vi "change channel select data typel test.vi"() -> ()   [LabVIEW 2015, in "tag select module tests.lvlib"]
uses:
  tag select module tests.lvlib
  module/configuration/tag select configuration.ctl
  <vilib>/NI/Tag Bus Module Framework/channel/TBM channel.lvclass
  <vilib>/NI/Tag Bus/tag/Data Type.ctl
  module/configuration/tag select module configuration.lvclass/tag select module configuration.ctl
  <vilib>/NI/Tag Bus/tag/tag descriptor.lvclass/tag descriptor.ctl
  module/configuration/Read tag select.vi
  <vilib>/NI/Tag Bus/tag/tag descriptor.lvclass
  module/configuration/tag select module configuration.lvclass
panel:
  out "data type 2":T1
  out "data type":T1
  out "data output 2":T1
  out "data select 2":T1
  out "data input A 2":T1
  out "data Input B 2":T1
  out "data Input B":T1
  out "data input A":T1
  out "data select":T1
  out "data output":T1
  out "input A 2":string
  out "input B 2":string
  out "input A":string
  out "input B":string
  out "select 2":string
  out "output 2":string
  out "select":string
  out "output":string
  out "tag select 2":T2[](array[typedef])
  out "tag select":T2[](array[typedef])
  out "no err":errorcluster
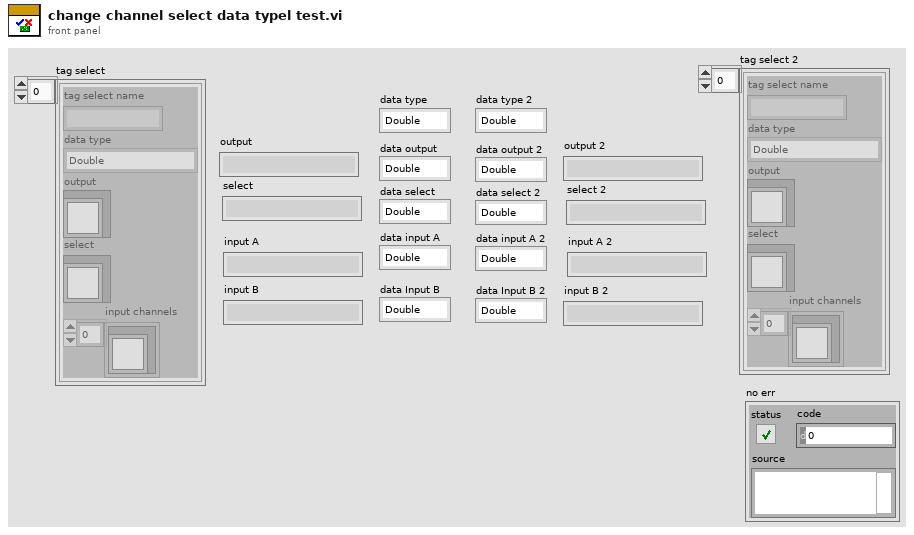
[diagram p1: front panel]
types:
  T1 = typedef "tag bus.lvlib/tag descriptor.lvclass/Data Type.ctl" = enum16{"Double", "Single", "I64", "I32", "I16", "I8", "U64", "U32", "U16", "U8", "Boolean", "String", "Array of Double", "Array of Single", "Array of I64", "Array of I32", "Array of I16", "Array of I8", "Array of U64", "Array of U32", "Array of U16", "Array of U8", "Array of Boolean", "Array of String"}
  T2 = typedef "tag select module configuration.lvclass/tag select configuration.ctl" = cluster{"tag select name":string, "data type":T1, "output":refnum<class "TBM channel.lvclass">, "select":refnum<class "TBM channel.lvclass">, "input channels":refnum<class "TBM channel.lvclass">[]}
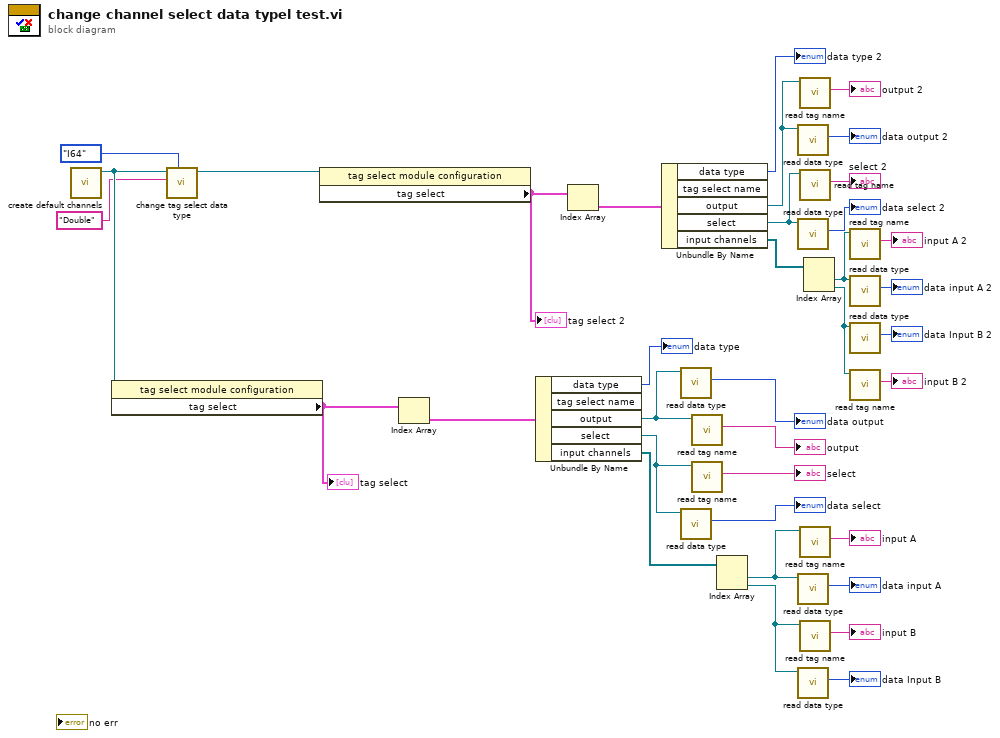
[diagram p0: block diagram]
diagram:
  n1 = call "create default channels.vi"() -> ("module"=w6:refnum<class "tag select module configuration.lvclass">)  [unwired: 8 in, 3 out]
  n2 = property class="tag select module configuration"(reference=w6) -> ("tag select"=w36:T2[])  [unwired: 1 in, 2 out]
  "tag select" <- w36
  n3 = call "change tag select data type.vi"("data type"=Data_Type."I64", "tag select name"="Double" ("old name"), "tag select  module configuration in"=w6) -> ("tag select module configuration out"=w5:refnum<class "tag select module configuration.lvclass">)  [unwired: 6 in, 2 out]
  n4 = property class="tag select module configuration"(reference=w5) -> ("tag select"=w29:T2[])  [unwired: 1 in, 2 out]
  "tag select 2" <- w29
  n5 = Index Array(array=w36) -> (element=w35:T2)  [unwired: 1 in]
  n6 = Unbundle By Name(w35) -> ("data type"=→"data type":T1, "output"=w15:refnum<class "TBM channel.lvclass">, "select"=w16:refnum<class "TBM channel.lvclass">, "input channels"=w28:refnum<class "TBM channel.lvclass">[])  [unwired: 1 out]
  n7 = Index Array(array=w29) -> (element=w32:T2)  [unwired: 1 in]
  n8 = Unbundle By Name(w32) -> ("data type"=→"data type 2":T1, "output"=w10:refnum<class "TBM channel.lvclass">, "select"=w9:refnum<class "TBM channel.lvclass">, "input channels"=w23:refnum<class "TBM channel.lvclass">[])  [unwired: 1 out]
  n9 = call <vilib>:"read data type.vi"("system tag in"=w15) -> ("data type"=→"data output":T1)  [unwired: 8 in, 2 out]
  n10 = call <vilib>:"read data type.vi"("system tag in"=w16) -> ("data type"=→"data select":T1)  [unwired: 8 in, 2 out]
  n11 = call <vilib>:"read tag name.vi"("system tag in"=w15) -> ("name"=→"output":string)  [unwired: 8 in, 2 out]
  n12 = call <vilib>:"read tag name.vi"("system tag in"=w16) -> ("name"=→"select":string)  [unwired: 8 in, 2 out]
  n13 = Index Array(array=w28) -> (element #1=w17:refnum<class "TBM channel.lvclass">, element #2=w18:refnum<class "TBM channel.lvclass">)  [unwired: 2 in]
  n14 = call <vilib>:"read data type.vi"("system tag in"=w10) -> ("data type"=→"data output 2":T1)  [unwired: 8 in, 2 out]
  n15 = call <vilib>:"read data type.vi"("system tag in"=w9) -> ("data type"=→"data select 2":T1)  [unwired: 8 in, 2 out]
  n16 = call <vilib>:"read data type.vi"("system tag in"=w17) -> ("data type"=→"data input A":T1)  [unwired: 8 in, 2 out]
  n17 = call <vilib>:"read data type.vi"("system tag in"=w18) -> ("data type"=→"data Input B":T1)  [unwired: 8 in, 2 out]
  n18 = call <vilib>:"read tag name.vi"("system tag in"=w10) -> ("name"=→"output 2":string)  [unwired: 8 in, 2 out]
  n19 = call <vilib>:"read tag name.vi"("system tag in"=w9) -> ("name"=→"select 2":string)  [unwired: 8 in, 2 out]
  n20 = call <vilib>:"read tag name.vi"("system tag in"=w17) -> ("name"=→"input A":string)  [unwired: 8 in, 2 out]
  n21 = call <vilib>:"read tag name.vi"("system tag in"=w18) -> ("name"=→"input B":string)  [unwired: 8 in, 2 out]
  n22 = Index Array(array=w23) -> (element #1=w8:refnum<class "TBM channel.lvclass">, element #2=w7:refnum<class "TBM channel.lvclass">)  [unwired: 2 in]
  n23 = call <vilib>:"read tag name.vi"("system tag in"=w8) -> ("name"=→"input A 2":string)  [unwired: 8 in, 2 out]
  n24 = call <vilib>:"read data type.vi"("system tag in"=w8) -> ("data type"=→"data input A 2":T1)  [unwired: 8 in, 2 out]
  n25 = call <vilib>:"read data type.vi"("system tag in"=w7) -> ("data type"=→"data Input B 2":T1)  [unwired: 8 in, 2 out]
  n26 = call <vilib>:"read tag name.vi"("system tag in"=w7) -> ("name"=→"input B 2":string)  [unwired: 8 in, 2 out]
